vi "RP1210 Client Disconnect.vi"(8 "error in (no error)":errorcluster, 11 "nClientID":i16) -> (0 "error out":errorcluster, 3 "function return":i16)   [LabVIEW 2020, in "cansub_rp1210.lvlib"]
doc: "short __stdcall RP1210_ClientDisconnect(short nClientID);"
uses:
  cansub_rp1210.lvlib
  cansub_lv64.dll
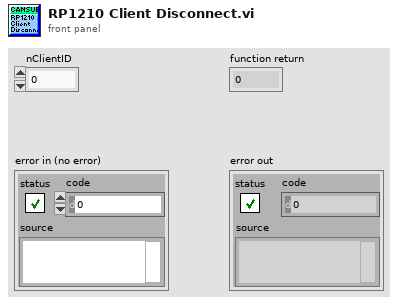
[diagram p1: front panel]
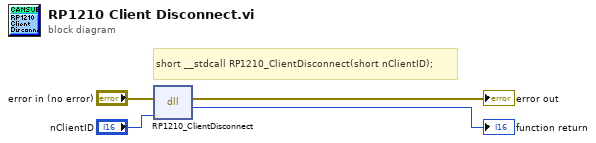
[diagram p0: block diagram]
diagram:
  # "short __stdcall RP1210_ClientDisconnect(short nClientID);"
  n1 = dll-call lib="C:/cansub-lv/library/cansub_lv*.*" fn="RP1210_ClientDisconnect"(error in="error in (no error)", "nClientID"="nClientID") -> (error out=→"error out":errorcluster, "return type"=→"function return":i16)  [unwired: 3 in, 1 out]
